vi "Unregister.vi"(8 "error in (no error)":errorcluster, 11 "logger name":string) -> (0 "error out":errorcluster, 3 "logger":refnum<class "Logger.lvclass">)   [LabVIEW 2018, in "GLog.lvlib" / "Registry.lvlib"]
uses:
  Registry.lvlib
  api/logger_class/Logger.lvclass
  Registry Actions.ctl
panel:
  # "Connector Pane"
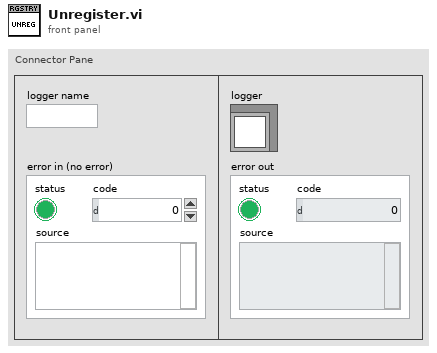
[diagram p1: front panel]
types:
  T1 = cluster{"Logging.lvlib:Logger.lvclass":refnum<class "Logger.lvclass">, "error in (no error)":errorcluster}
  T2 = typedef "GLog.lvlib/Registry.lvlib/Registry Actions.ctl" = enum16{"Register", "Log", "Enable", "Enable All", "Disable", "Disable All", "Get Enable State", "Get Minimum Log Level", "Set Minimum Log Level", "Set All Minimum Log Level", "Get Logger Info", "Get All Logger Info", "List", "Unregister", "Unregister All", "Shutdown"}
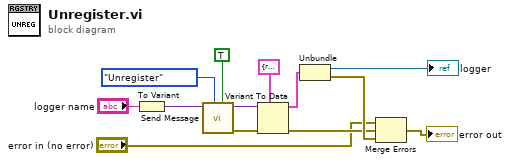
[diagram p0: block diagram]
diagram:
  n1 = To Variant(anything="logger name") -> (Variant=w12:variant)
  n2 = call "Send Message.vi"("return data? (F)"=TRUE, "action"=Registry_Actions."Unregister", "send data"=w12) -> ("error out"=w3:errorcluster, "Variant"=w11:variant)  [unwired: 7 in]
  n3 = Variant To Data(error in=w3, type=T1 {"Logging.lvlib:Logger.lvclass"=refnum, "error in (no error)"={"status"=FALSE, "code"=0, "source"=""}}, Variant=w11) -> (data=w6:T1, error out=w2:errorcluster)
  n4 = Unbundle(w6) -> ("Logging.lvlib:Logger.lvclass"=→"logger":refnum<class "Logger.lvclass">, "error in (no error)"=w4:errorcluster)
  n5 = Merge Errors("error in (no error)", w2, w4) -> (→"error out":errorcluster)
